vi "TCP Server Example Connection Handler VI.vi"(9 "Additional Data":variant, 10 "connection ID":T1, 11 "TCP Server Refnum":refnum<class "JKI TCP Server.lvclass">) -> ()   [LabVIEW 2020]
uses:
  _Data Structures/TCP Server Connection Session ID Cluster.ctl
  JKI TCP Server.lvclass
panel:
  # "Copyright © 2004-2008 JKI. All rights reserved.\n\nAuthor: Jim Kring [jim.kring@jameskring.com]\n\nThis library is provided \"AS IS\" ,WITHOUT WARRANTIES OR \nCONDITIONS OF ANY KIND, either express or implied.\n\nJames Kring, Inc. -- http://www.jameskring.com"
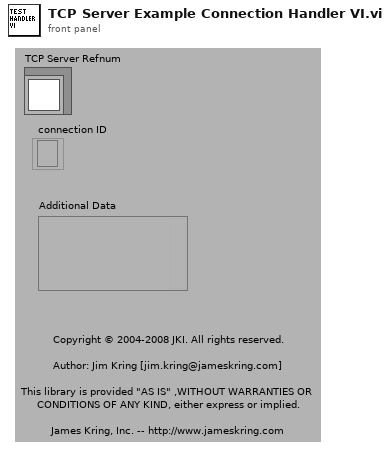
[diagram p1: front panel]
types:
  T1 = typedef "JKI TCP Server.lvclass/TCP Server Connection Session ID Cluster.ctl" = refnum<k5>
  T2 = enum16{"Standard", "Buffered", "CRLF", "Immediate"}
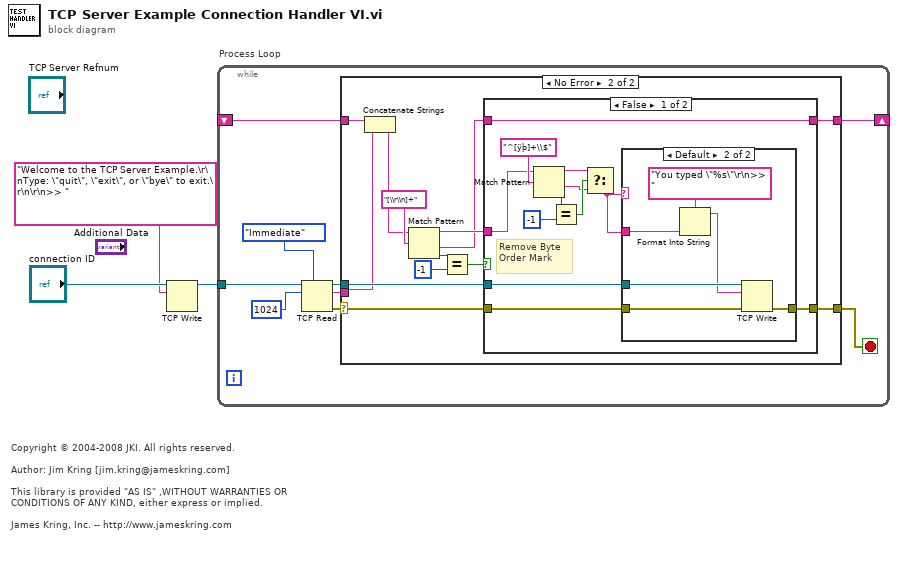
[diagram p0: block diagram]
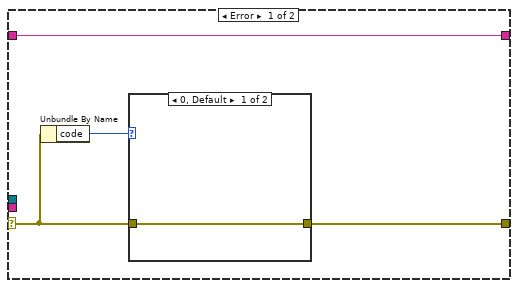
[diagram p2: hidden frame]
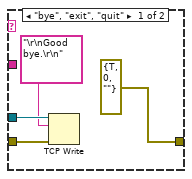
[diagram p4: hidden frame]
diagram:
  # "Copyright © 2004-2008 JKI. All rights reserved.\n\nAuthor: Jim Kring [jim.kring@jameskring.com]\n\nThis library is provided \"AS IS\" ,WITHOUT WARRANTIES OR \nCONDITIONS OF ANY KIND, either express or implied.\n\nJames Kring, Inc. -- http://www.jameskring.com"
  n1 = TCP Write(connection ID="connection ID", data in="Welcome to the TCP Server Example.\r\nType: \"quit\", \"exit\", or \"bye\" to exit.\r\n\r\n>> ") -> (connection ID out=w2:T1)  [unwired: 2 in, 2 out]
  n2 = while "Process Loop" {
    tunnel: w2 -> [w7]
    shift-right: [w5] -> _
    shift-left: _ -> [w6]
    stop <- w12 stop-if-true
    n3 = TCP Read(connection ID=w7, bytes to read=1024, 7:T2."Immediate" ("mode (standard)")) -> (connection ID out=w8:T1, data out=w9:string, error out=w10:errorcluster)  [unwired: 2 in]
    n4 = case shown="No Error" w10 {
      selector: w10 -> [w15 w27]
      tunnel: w8 -> [_ w30]
      tunnel: w9 -> [_ w21]
      tunnel: [w14 w28] -> w12
      tunnel: w6 -> [w13 w22]
      tunnel: [w13 w18] -> w5
      frame Error {
        n5 = Unbundle By Name(w15) -> ("code"=w16:i32)
        n6 = case shown="0, Default" w16 {
          tunnel: w15 -> [w17 _]
          tunnel: [w17 _] -> w14
          frame 0, Default {
          }
          frame 56 {
          }
        }
      }
      frame No Error {
        n7 = Concatenate Strings(w22, w21) -> (w20:string)
        n8 = Match Pattern(string=w20, regular expression="[\\r\\n]+") -> (before substring=w26:string, after substring=w19:string, offset past match=w25:i32)  [unwired: 1 in, 1 out]
        n9 = Equal?(x=w25, y=-1) -> (x = y?=w23:bool)
        n10 = case shown="False" w23 {
          tunnel: w30 -> [w42 _]
          tunnel: [w41 w53] -> w28
          tunnel: w27 -> [w40 w53]
          tunnel: w26 -> [w31 w54]
          tunnel: w19 -> [w39 _]
          tunnel: [w39 w54] -> w18
          frame False {
            # "Remove Byte Order Mark"
            n11 = Match Pattern(string=w31, regular expression="^[ÿþ]+\\$") -> (before substring=w34:string, after substring=w33:string, offset past match=w36:i32)  [unwired: 1 in, 1 out]
            n12 = Equal?(x=w36, y=-1) -> (x = y?=w35:bool)
            n13 = Select(t=w34, s=w35, f=w33) -> (s? t:f=w32:string)
            n14 = case shown="Default" w32 {
              tunnel: w42 -> [w44 w52]
              tunnel: [errorcluster {"status"=TRUE, "code"=0, "source"=""} ("error out") w49] -> w41
              tunnel: w40 -> [w45 w48]
              tunnel: w32 -> [_ w47]
              frame "bye", "exit", "quit" {
                n15 = TCP Write(connection ID=w44, data in="\r\nGood bye.\r\n", error in (no error)=w45) -> ()  [unwired: 1 in, 3 out]
              }
              frame Default {
                n16 = Format Into String(format string="You typed \"%s\"\r\n>> ", w47) -> (resulting string=w50:string)  [unwired: 2 in, 1 out]
                n17 = TCP Write(connection ID=w52, data in=w50, error in (no error)=w48) -> (error out=w49:errorcluster)  [unwired: 1 in, 2 out]
              }
            }
          }
          frame True {
          }
        }
      }
    }
  }
